vi "Cmd_JogWord.vi"(8 "Masks":string[](array[string]), 9 "Prev":bool[](array[boolean]), 10 "Bits":bool[](array[boolean]), 11 "Queue":refnum<queue>) -> ()   [LabVIEW 2026]
doc: "Use this template to build a VI to use as a subVI."
panel:
  # "ÕfÃ÷£ºÊÖ„Ó°´âoÓÐ×ƒ„Ó•r£¬°ÑÈ«²¿°´âo½M³ÉÒ»‚€×ÖŒ‘µ½ D107¡£·Åé_•rŒ‘\n»Ø 0¡£"
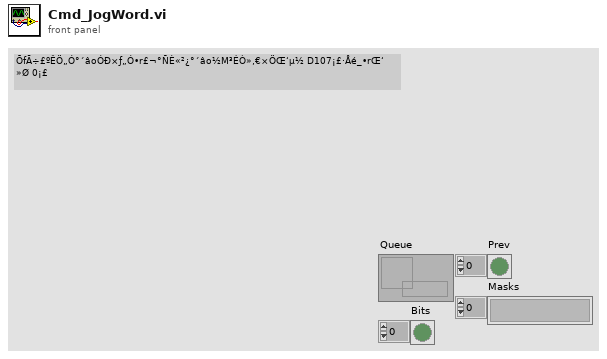
[diagram p1: front panel]
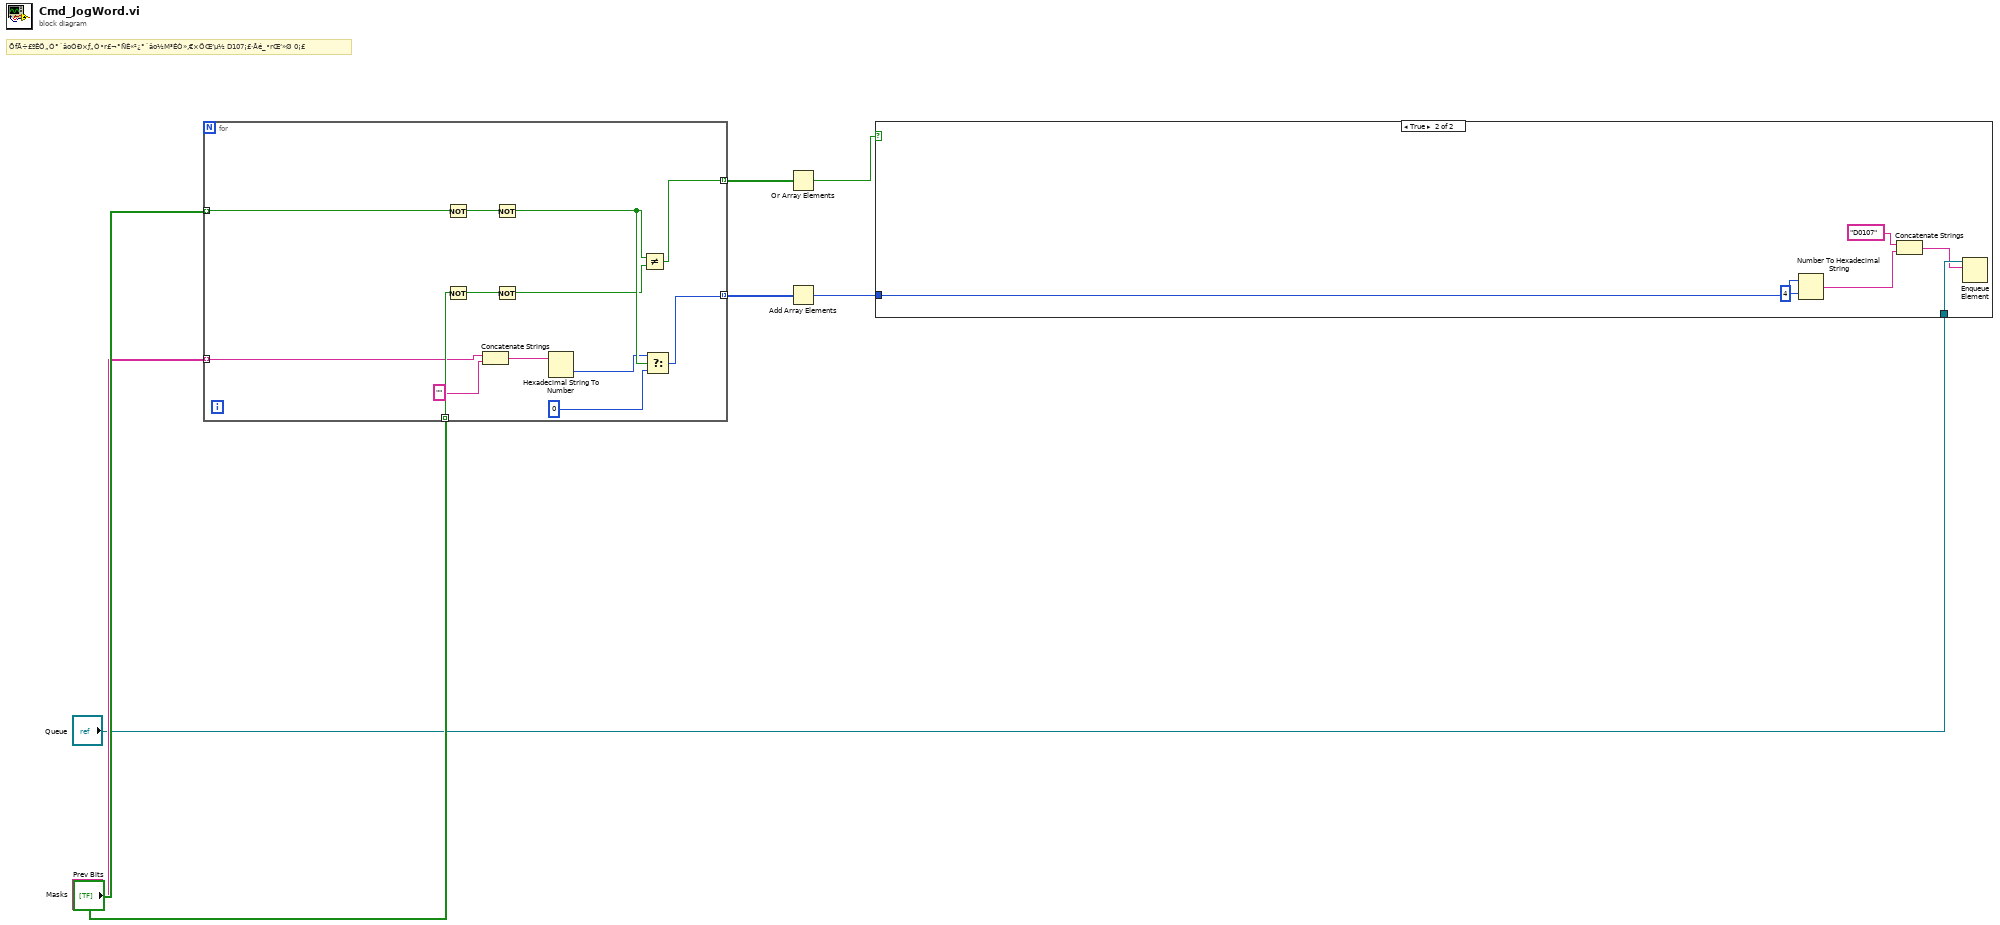
[diagram p0: block diagram]
diagram:
  # "ÕfÃ÷£ºÊÖ„Ó°´âoÓÐ×ƒ„Ó•r£¬°ÑÈ«²¿°´âo½M³ÉÒ»‚€×ÖŒ‘µ½ D107¡£·Åé_•rŒ‘»Ø 0¡£"
  n1 = for {
    tunnel: "Bits" -> [w21] mode=indexing
    tunnel: "Prev" -> [w19] mode=indexing
    tunnel: "Masks" -> [w17] mode=indexing
    tunnel: [w10] -> w5 mode=indexing
    tunnel: [w9] -> w4 mode=indexing
    n2 = Not(x=w21) -> (.not. x?=w20:bool)
    n3 = Not(x=w19) -> (.not. x?=w18:bool)
    n4 = Concatenate Strings(w17, "") -> (w15:string)
    n5 = Not(x=w20) -> (.not. x?=w14:bool)
    n6 = Not(x=w18) -> (.not. x?=w11:bool)
    n7 = Hexadecimal String To Number(string=w15) -> (number=w13:u32)  [unwired: 2 in, 1 out]
    n8 = Not Equal?(x=w14, y=w11) -> (x != y?=w9:bool)
    n9 = Select(t=w13, s=w14, f=0) -> (s? t:f=w10:u32)
  }
  n10 = Or Array Elements(Boolean array=w4) -> (logical OR=w3:bool)
  n11 = Add Array Elements(numeric array=w5) -> (sum=w2:u32)
  n12 = case shown="True" w3 {
    tunnel: w2 -> [_ w27]
    tunnel: "Queue" -> [_ w23]
    frame False {
    }
    frame True {
      n13 = Number To Hexadecimal String(1:i16 4 ("width (-)"), 2:w27) -> (0:w24:string)
      n14 = Concatenate Strings("D0107", w24) -> (w22:string)
      n15 = Enqueue Element(queue=w23, element=w22) -> ()  [unwired: 2 in, 3 out]
    }
  }
